vi "write WatchDog.vi"(9 "data":variant, 10 "station":string, 11 "URL":string) -> (3 "ok?":bool)   [LabVIEW 2012]
uses:
  Globals/Global.vi
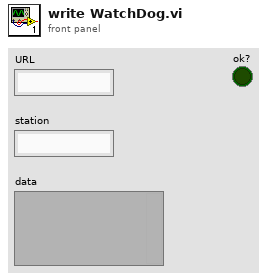
[diagram p1: front panel]
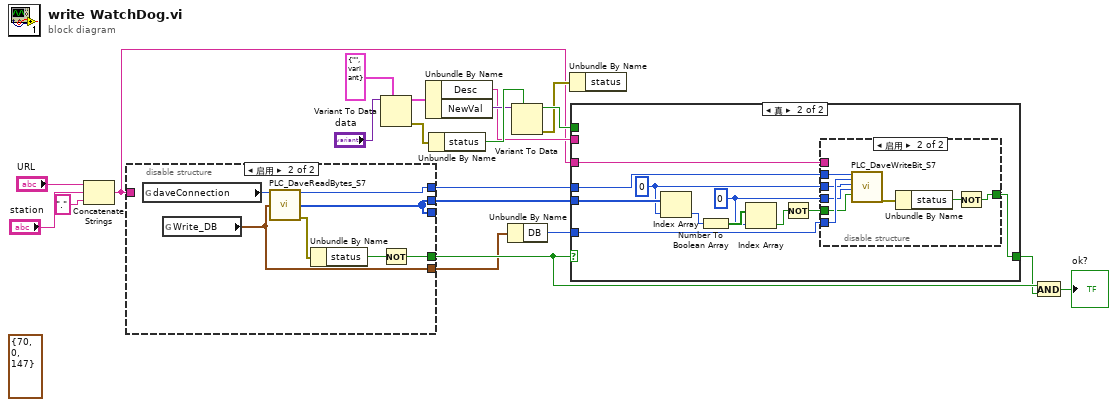
[diagram p0: block diagram]
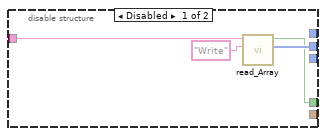
[diagram p2: hidden frame]
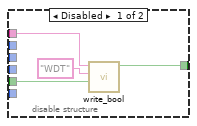
[diagram p4: hidden frame]
diagram:
  (unwired) cluster{"DB":i32, "start":i32, "len":i32} {"DB"=70, "start"=0, "len"=147} ("地址")
  n1 = Concatenate Strings("URL", "station", "." ("string")) -> (w7:string)
  n2 = disable-structure shown="启用" {
    disable-tunnel: [w24 w30] -> w10
    disable-tunnel: w7 -> [w23 _]
    disable-tunnel: [w21 w26] -> w6
    disable-tunnel: [_ w30] -> _
    disable-tunnel: [_ w29] -> w3
    disable-tunnel: [_ w25] -> w2
    frame Disabled {
      n3 = call "read_Array.vi"("Address"="Write", "URL"=w23) -> ("Value"=w24:u8[], "ok?"=w21:bool)  [unwired: 7 in, 1 out]
    }
    frame Enabled {
      n4 = global read "Global.vi" "daveConnection"() -> (w31:i64)
      n5 = global read "Global.vi" "Write_DB"() -> (w25:cluster{"DB":i32, "start":i32, "len":i32})
      n6 = call "PLC_DaveReadBytes_S7.vi"("daveConnection in"=w31, "地址"=w25) -> ("daveConnection out"=w29:i64, "read Buffer"=w30:u8[], "error out"=w27:errorcluster)  [unwired: 10 in, 1 out]
      n7 = Unbundle By Name(w27) -> ("status"=w28:bool)
      n8 = Not(x=w28) -> (.not. x?=w26:bool)
    }
  }
  n9 = Variant To Data(type=cluster{"Desc":string, "NewVal":variant} {"Desc"="", "NewVal"=variant} ("output cluster"), Variant="data") -> (data=w14:cluster{"Desc":string, "NewVal":variant}, error out=w12:errorcluster)  [unwired: 1 in]
  n10 = Unbundle By Name(w14) -> ("Desc"=w15:string, "NewVal"=w16:variant)
  n11 = Unbundle By Name(w12) -> ("status"=w17:bool)
  n12 = Unbundle By Name(w2) -> ("DB"=w1:i32)
  n13 = Variant To Data(type=w17, Variant=w16) -> (data=w19:bool, error out=w18:errorcluster)  [unwired: 1 in]
  n14 = Unbundle By Name(w18) -> ()  [unwired: 1 out]
  n15 = case shown="真" w6 {
    selector: w6 -> [w32 _]
    tunnel: w7 -> [_ w39]
    tunnel: w10 -> [_ w43]
    tunnel: w19 -> [_ _]
    tunnel: w15 -> [_ _]
    tunnel: [w32 w37] -> w4
    tunnel: w3 -> [_ w36]
    tunnel: w1 -> [_ w35]
    frame False {
    }
    frame True {
      w33 = 0 ("index")
      w34 = 0 ("index")
      n16 = Index Array(array=w43, index=w34) -> (element=w42:u8)
      n17 = Number To Boolean Array(number=w42) -> (Boolean array=w41:bool[])
      n18 = Index Array(array=w41, index=w33) -> (element=w40:bool)
      n19 = Not(x=w40) -> (.not. x?=w38:bool)
      n20 = disable-structure shown="启用" {
        disable-tunnel: w39 -> [w47 _]
        disable-tunnel: w38 -> [w45 w51]
        disable-tunnel: [w44 w48] -> w37
        disable-tunnel: w36 -> [_ w55]
        disable-tunnel: w35 -> [_ w54]
        disable-tunnel: w34 -> [_ w53]
        disable-tunnel: w33 -> [_ w52]
        frame Disabled {
          n21 = call "write_bool.vi"("Value"=w45, "Address"="WDT", "URL"=w47) -> ("ok?"=w44:bool)  [unwired: 7 in, 1 out]
        }
        frame Enabled {
          n22 = call "PLC_DaveWriteBit_S7.vi"("daveConnection IN"=w55, "DB"=w54, "byte"=w53, "bit"=w52, "value"=w51) -> ("error out"=w50:errorcluster)  [unwired: 12 in, 2 out]
          n23 = Unbundle By Name(w50) -> ("status"=w49:bool)
          n24 = Not(x=w49) -> (.not. x?=w48:bool)
        }
      }
    }
  }
  n25 = And(x=w6, y=w4) -> (x .and. y?=→"ok?":bool)
